vi "Write String.vi"(8 "error in (no error)":errorcluster, 9 "offset (0)":i64, 10 "string in":string, 11 "pointer in":u64) -> (0 "error out":errorcluster, 1 "offset out":i64, 2 "bytes written":i64, 3 "pointer out":u64)   [LabVIEW 2016, in "Linux RT IPC.Shared Memory.lvlib"]
uses:
  Linux RT IPC.Shared Memory.lvlib
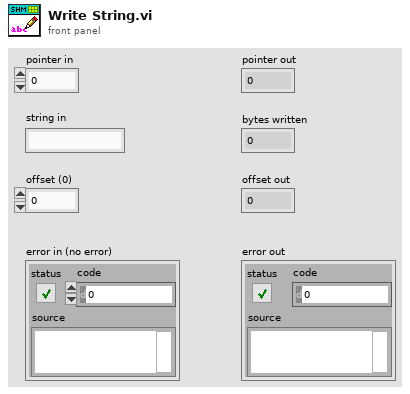
[diagram p1: front panel]
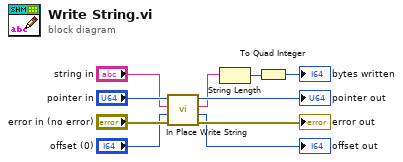
[diagram p0: block diagram]
diagram:
  n1 = call "In Place Write String.vi"("error in (no error)"="error in (no error)", "offset (0)"="offset (0)", "string in"="string in", "pointer in"="pointer in") -> ("error out"=→"error out":errorcluster, "offset out"=→"offset out":i64, "string out"=w2:string, "pointer out"=→"pointer out":u64)  [unwired: 4 in]
  n2 = String Length(string=w2) -> (length=w3:i32)
  n3 = To Quad Integer(1:w3) -> (0:→"bytes written":i64)
